vi "VOLTAGE.vi"(9 "INPUT VOLTAGE":dbl) -> (3 "voltage output":dbl)   [LabVIEW 2016]
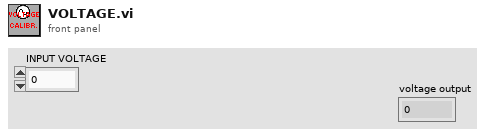
[diagram p1: front panel]
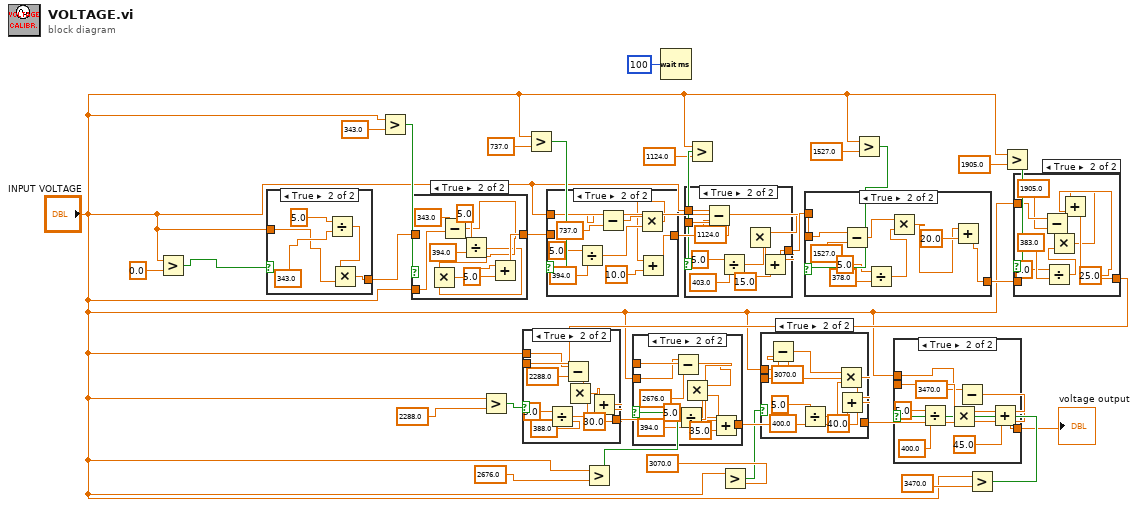
[diagram p0: block diagram]
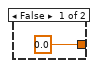
[diagram p11: hidden frame]
diagram:
  n1 = Greater?(x="INPUT VOLTAGE", y=0.0) -> (0:w32:bool)
  n2 = case shown="True" w32 {
    tunnel: [0.0 ("y") w37] -> w12
    tunnel: "INPUT VOLTAGE" -> [_ w34]
    frame False {
    }
    frame True {
      n3 = Divide(x=5.0 ("y"), y=343.0) -> (x/y=w38:dbl)
      n4 = Multiply(x=w38, y=w34) -> (x*y=w37:dbl)
    }
  }
  n5 = Greater?(x="INPUT VOLTAGE", y=343.0) -> (0:w29:bool)
  n6 = case shown="True" w29 {
    tunnel: w12 -> [w39 _]
    tunnel: [w39 w48] -> w26
    tunnel: "INPUT VOLTAGE" -> [_ w45]
    frame False {
    }
    frame True {
      n7 = Subtract(x=w45, y=343.0) -> (x-y=w42:dbl)
      n8 = Divide(x=5.0, y=394.0) -> (x/y=w41:dbl)
      n9 = Multiply(x=w42, y=w41) -> (x*y=w40:dbl)
      n10 = Add(x=w40, y=5.0) -> (x+y=w48:dbl)
    }
  }
  n11 = Greater?(x="INPUT VOLTAGE", y=2288.0) -> (0:w14:bool)
  n12 = Greater?(x="INPUT VOLTAGE", y=737.0) -> (0:w27:bool)
  n13 = case shown="True" w27 {
    tunnel: [w49 w57] -> w25
    tunnel: w26 -> [w49 _]
    tunnel: "INPUT VOLTAGE" -> [_ w55]
    frame False {
    }
    frame True {
      n14 = Divide(x=5.0, y=394.0) -> (x/y=w51:dbl)
      n15 = Subtract(x=w55, y=737.0) -> (x-y=w52:dbl)
      n16 = Multiply(x=w52, y=w51) -> (x*y=w50:dbl)
      n17 = Add(x=w50, y=10.0) -> (x+y=w57:dbl)
    }
  }
  n18 = Greater?(x="INPUT VOLTAGE", y=2676.0) -> (0:w10:bool)
  n19 = Wait (ms)(milliseconds to wait=u32 100) -> ()  [unwired: 1 out]
  n20 = Greater?(x="INPUT VOLTAGE", y=1124.0) -> (0:w24:bool)
  n21 = case shown="True" w24 {
    tunnel: w25 -> [w59 _]
    tunnel: "INPUT VOLTAGE" -> [_ w67]
    tunnel: [w59 w65] -> w21
    frame False {
    }
    frame True {
      n22 = Subtract(x=w67, y=1124.0) -> (x-y=w62:dbl)
      n23 = Divide(x=5.0, y=403.0) -> (x/y=w61:dbl)
      n24 = Multiply(x=w62, y=w61) -> (x*y=w60:dbl)
      n25 = Add(x=w60, y=15.0) -> (x+y=w65:dbl)
    }
  }
  n26 = Greater?(x="INPUT VOLTAGE", y=3070.0) -> (0:w6:bool)
  n27 = Greater?(x="INPUT VOLTAGE", y=1527.0) -> (0:w20:bool)
  n28 = case shown="True" w20 {
    tunnel: [w69 w75] -> w17
    tunnel: w21 -> [w69 _]
    tunnel: "INPUT VOLTAGE" -> [_ w77]
    frame False {
    }
    frame True {
      n29 = Subtract(x=w77, y=1527.0) -> (x-y=w71:dbl)
      n30 = Divide(x=5.0, y=378.0) -> (x/y=w73:dbl)
      n31 = Multiply(x=w71, y=w73) -> (x*y=w70:dbl)
      n32 = Add(x=w70, y=20.0) -> (x+y=w75:dbl)
    }
  }
  n33 = Greater?(x="INPUT VOLTAGE", y=3470.0) -> (0:w5:bool)
  n34 = Greater?(x="INPUT VOLTAGE", y=1905.0) -> (0:w18:bool)
  n35 = case shown="True" w18 {
    tunnel: [w79 w85] -> w15
    tunnel: w17 -> [w79 _]
    tunnel: "INPUT VOLTAGE" -> [_ w88]
    frame False {
    }
    frame True {
      n36 = Subtract(x=w88, y=1905.0) -> (x-y=w81:dbl)
      n37 = Divide(x=5.0, y=383.0) -> (x/y=w82:dbl)
      n38 = Multiply(x=w81, y=w82) -> (x*y=w80:dbl)
      n39 = Add(x=w80, y=25.0) -> (x+y=w85:dbl)
    }
  }
  n40 = case shown="True" w14 {
    tunnel: [w89 w95] -> w13
    tunnel: "INPUT VOLTAGE" -> [_ w96]
    tunnel: w15 -> [w89 _]
    frame False {
    }
    frame True {
      n41 = Divide(x=5.0, y=388.0) -> (x/y=w92:dbl)
      n42 = Subtract(x=w96, y=2288.0) -> (x-y=w91:dbl)
      n43 = Multiply(x=w91, y=w92) -> (x*y=w90:dbl)
      n44 = Add(x=w90, y=30.0) -> (x+y=w95:dbl)
    }
  }
  n45 = case shown="True" w10 {
    tunnel: [w99 w104] -> w9
    tunnel: w13 -> [w99 _]
    tunnel: "INPUT VOLTAGE" -> [_ w106]
    frame False {
    }
    frame True {
      n46 = Subtract(x=w106, y=2676.0) -> (x-y=w101:dbl)
      n47 = Divide(x=5.0, y=394.0) -> (x/y=w100:dbl)
      n48 = Multiply(x=w101, y=w100) -> (x*y=w102:dbl)
      n49 = Add(x=w102, y=35.0) -> (x+y=w104:dbl)
    }
  }
  n50 = case shown="True" w6 {
    tunnel: [w109 w114] -> w8
    tunnel: w9 -> [w109 _]
    tunnel: "INPUT VOLTAGE" -> [_ w117]
    frame False {
    }
    frame True {
      n51 = Subtract(x=w117, y=3070.0) -> (x-y=w113:dbl)
      n52 = Divide(x=5.0, y=400.0) -> (x/y=w112:dbl)
      n53 = Multiply(x=w113, y=w112) -> (x*y=w110:dbl)
      n54 = Add(x=w110, y=40.0) -> (x+y=w114:dbl)
    }
  }
  n55 = case shown="True" w5 {
    tunnel: [w119 w124] -> w3
    tunnel: w8 -> [w119 _]
    tunnel: "INPUT VOLTAGE" -> [_ w126]
    frame False {
    }
    frame True {
      n56 = Divide(x=5.0, y=400.0) -> (x/y=w121:dbl)
      n57 = Subtract(x=w126, y=3470.0) -> (x-y=w122:dbl)
      n58 = Multiply(x=w122, y=w121) -> (x*y=w120:dbl)
      n59 = Add(x=w120, y=45.0) -> (x+y=w124:dbl)
    }
  }
  "voltage output" <- w3
